vi "Test Process within App Log Info Message.vi"(8 "error in (no error)":errorcluster, 11 "Test Case In":refnum<class "Logger Test.lvclass">) -> (0 "error out":errorcluster, 3 "Test Case Out":refnum<class "Logger Test.lvclass">)   [LabVIEW 2020, in "Logger Test.lvclass"]
uses:
  Logger Test.lvclass
  C:/Program Files (x86)/National Instruments/LabVIEW 2020/vi.lib/Astemes/LUnit/Test Case.lvclass
  source/Framework Test Suite/Mock Log Handler/Mock Log Handler.lvclass
  C:/git/astemes-triarc-framework/source/Framework/Logging/Logging.lvclass
  source/Framework/Application/Application.lvclass
  C:/git/astemes-triarc-framework/source/Framework/Process/Process.lvclass
  source/Framework Test Suite/Mock Process/Mock Process.lvclass
  source/Framework/Process/Process.lvclass/Process.ctl
  source/Framework/Application/Application.lvclass/Application.ctl
  <vilib>/Astemes/LUnit/Test Case.lvclass/Test Case.ctl
  79509b29-02db-4acb-a020-dc3c62102361.vi
  1ed042bb-7d1b-42fa-8c49-f08837779b5c.vi
  d456e797-6803-49a2-97fa-78168cfad702.vi
  source/Framework/Process/Public/Lifecycle/Get Lifecycle State.vi
  source/Framework/Process/Protected/Messaging/Send Message.vi
  source/Framework/Application/Private/Add Process to Map.vi
  source/Framework/Application/Private/Throw Error If Process Already in App.vi
  source/Framework/Process/Protected/SubVIs/Set Context.vi
  source/Framework/Process/Private/SubVIs/Wait for finish.vi
  source/Framework/Process/Private/SubVIs/Set Lifecycle State.vi
  <vilib>/Astemes/LUnit/Append Pass Result.vi
  <vilib>/Astemes/LUnit/Append Fail Result.vi
  <vilib>/Astemes/LUnit/Describe Comparison.vi
  <vilib>/Astemes/LUnit/Compare Variants.vi
  source/Framework/Process/Private/SubVIs/Handle Debug Data.vi
  source/Framework/Application/Public/Get Process.vi
  <vilib>/Astemes/LUnit/Variant to string.vi
  source/Framework/Logging/Log Debug.vi
  <vilib>/AdvancedString/1D String Array to Delimited String.vi
  <vilib>/Utility/High Resolution Relative Seconds.vi
  source/Framework/Application/Private/Retrieve Process from App.vi
  source/Framework/Application/Private/Parse Process Name.vi
  source/Framework/Application/Private/Get Process from Map.vi
  source/Framework/Process/Protected/Messaging/Request Message.vi
  <vilib>/AdvancedString/Delimited String to 1D String Array.vi
  source/Framework/Process/Private/SubVIs/Enqueue Request Message.vi
  source/Framework/Process/Process.lvclass
  source/Framework/Process/Public/Read Name.vi
  <vilib>/Utility/error.llb/Error Cluster From Error Code.vi
  source/Framework/Process/Private/SubVIs/Wait for Response Message.vi
  <vilib>/Utility/Data Type/Get Type Information.vi
  <vilib>/Utility/LVClass/Get LV Class Name.vi
  source/Framework/Logging/Logging.lvclass
  Logger Test.lvclass/Logger Test.ctl
  source/Framework Test Suite/Support/Test Support.lvlib
  C:/git/astemes-triarc-framework/source/Framework/Base/Base.lvclass
  C:/git/astemes-triarc-framework/source/Framework/Error Handler Interface/Error Handler Interface.lvclass
  C:/git/astemes-triarc-framework/source/Framework/Application/Application.lvclass
  C:/git/astemes-triarc-framework/source/Framework/Async Handler/Async Handler.lvclass
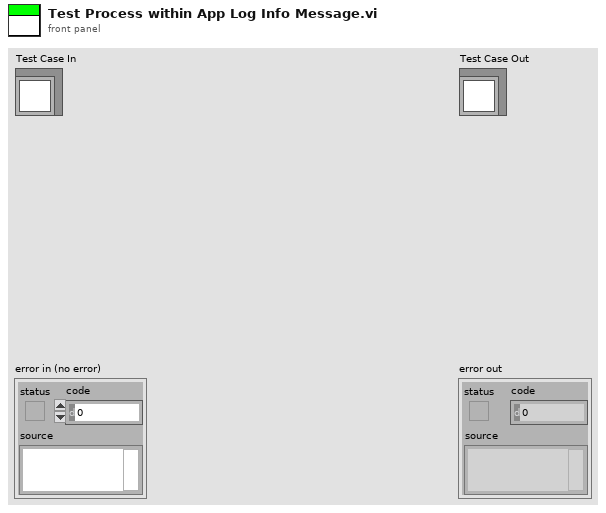
[diagram p1: front panel]
types:
  T1 = typedef "Mock Log Handler.lvclass/Log Entry.ctl" = cluster{"Level":string, "Source":string, "Message":string}
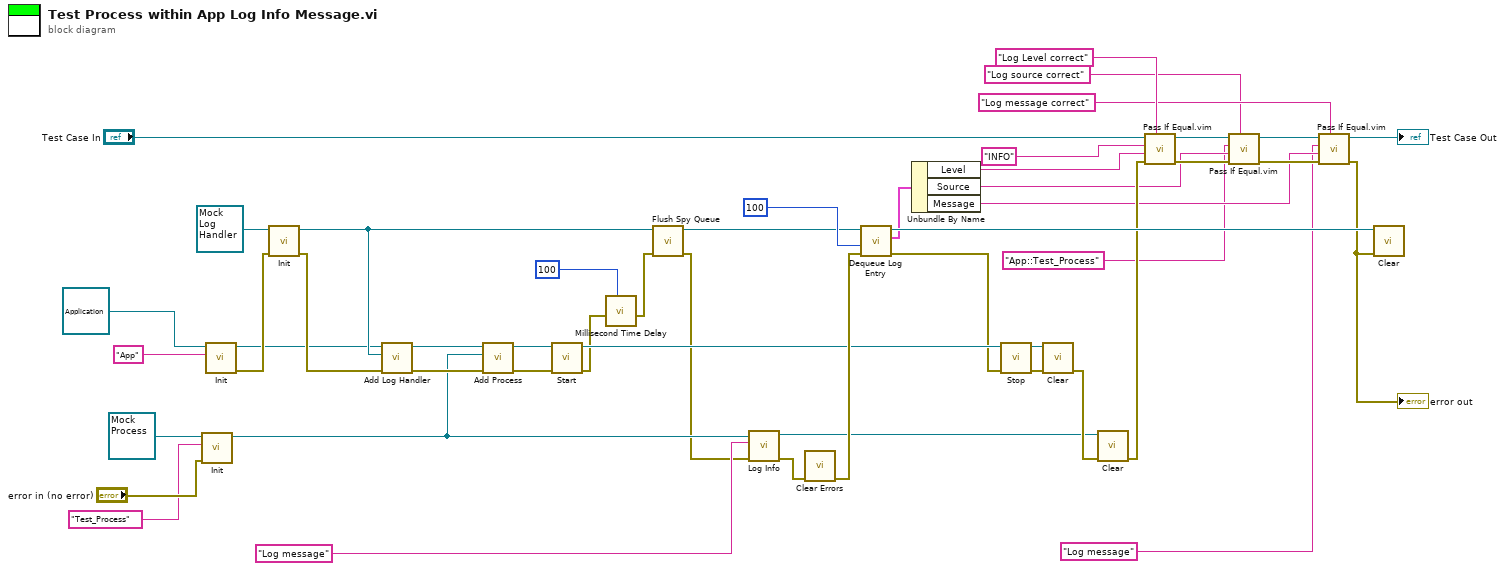
[diagram p0: block diagram]
diagram:
  n1 = call-dynamic "Init.vi"("error in (no error)"="error in (no error)", "Name"="Test_Process", "Mock Process In"=refnum<class "Mock Process.lvclass"> refnum) -> ("Mock Process Out"=w6:refnum<class "Mock Process.lvclass">)  [unwired: 7 in, 1 out]
  n2 = call-dynamic "Init.vi"("Name"="App", "Process In"=refnum<class "Application.lvclass"> refnum ("Application.lvclass")) -> ("error out"=w44:errorcluster, "Process Out"=w4:refnum<class "Application.lvclass">)  [unwired: 8 in]
  n3 = call-dynamic "Init.vi"("error in (no error)"=w44, "Mock Log Handler In"=refnum<class "Mock Log Handler.lvclass"> refnum ("Mock Log Handler.lvclass")) -> ("error out"=w43:errorcluster, "Mock Log Handler Out"=w11:refnum<class "Mock Log Handler.lvclass">)  [unwired: 8 in]
  n4 = call "Add Log Handler.vi"("error in (no error)"=w43, "Log Handler"=w11, "Process In"=w4) -> ("error out"=w21:errorcluster, "Process Out"=w20:refnum<class "Application.lvclass">)  [unwired: 7 in]
  n5 = call "Add Process.vi"("error in (no error)"=w21, "Process"=w6, "Application In"=w20) -> ("error out"=w17:errorcluster, "Application Out"=w3:refnum<class "Application.lvclass">)  [unwired: 7 in]
  n6 = call "Start.vi"("error in (no error)"=w17, "Process In"=w3) -> ("error out"=w9:errorcluster, "Process Out"=w13:refnum<class "Application.lvclass">)  [unwired: 7 in, 1 out]
  n7 = call "Millisecond Time Delay.vi"("milliseconds to wait"=u32 100, "error in (no error)"=w9) -> ("error out"=w8:errorcluster)  [unwired: 7 in]
  n8 = call "Flush Spy Queue.vi"("error in (no error)"=w8, "Mock Log Handler in"=w11) -> ("error out"=w5:errorcluster, "Mock Log Handler out"=w10:refnum<class "Mock Log Handler.lvclass">)  [unwired: 7 in, 1 out]
  n9 = call "Log Info.vi"("error in (no error)"=w5, "Message"="Log message", "Logging In"=w6) -> ("error out"=w27:errorcluster, "Logging Out"=w14:refnum<class "Mock Process.lvclass">)  [unwired: 7 in]
  n10 = call <vilib>:"Clear Errors.vi"("error in (no error)"=w27) -> ("error out"=w26:errorcluster)  [unwired: 5 in, 1 out]
  n11 = call "Dequeue Log Entry.vi"("error in (no error)"=w26, "timeout in ms (-1)"=100, "Mock Log Handler in"=w10) -> ("error out"=w2:errorcluster, "Entry"=w40:T1, "Mock Log Handler out"=w42:refnum<class "Mock Log Handler.lvclass">)  [unwired: 5 in, 1 out]
  n12 = Unbundle By Name(w40) -> ("Level"=w39:string, "Source"=w30:string, "Message"=w29:string)
  n13 = call "Stop.vi"("error in (no error)"=w2, "Process In"=w13) -> ("error out"=w16:errorcluster, "Process Out"=w15:refnum<class "Application.lvclass">)  [unwired: 7 in, 1 out]
  n14 = call-dynamic "Clear.vi"("error in (no error)"=w16, "Application In"=w15) -> ("error out"=w46:errorcluster)  [unwired: 9 in]
  n15 = call-dynamic "Clear.vi"("error in (no error)"=w46, "Mock Process In"=w14) -> ("error out"=w33:errorcluster)  [unwired: 9 in]
  n16 = call "Pass If Equal.vim"("Description"="Log Level correct", "error in (no error)"=w33, "Actual"=w39, "Expected"="INFO", "LUnit Test Case In"="Test Case In") -> ("error out"=w35:errorcluster, "LUnit Test Case Out"=w48:refnum<class "Logger Test.lvclass">)  [unwired: 5 in]
  n17 = call "Pass If Equal.vim"("Description"="Log source correct", "error in (no error)"=w35, "Actual"=w30, "Expected"="App::Test_Process" ("Name"), "LUnit Test Case In"=w48) -> ("error out"=w34:errorcluster, "LUnit Test Case Out"=w37:refnum<class "Logger Test.lvclass">)  [unwired: 5 in]
  n18 = call "Pass If Equal.vim"("Description"="Log message correct", "error in (no error)"=w34, "Actual"=w29, "Expected"="Log message" ("Message"), "LUnit Test Case In"=w37) -> ("error out"=w1:errorcluster, "LUnit Test Case Out"=→"Test Case Out":refnum<class "Logger Test.lvclass">)  [unwired: 5 in]
  "error out" <- w1
  n19 = call-dynamic "Clear.vi"("error in (no error)"=w1, "Mock Log Handler In"=w42) -> ()  [unwired: 9 in, 1 out]
